vi "VIH Utility - FILE - List Directory Advanced.vi"(4 "Exclude Dir patterns":string[](array[string]), 6 "Exclude File patterns":string[](array[string]), 7 "List recursively (F)":bool, 8 "error in":errorcluster, 9 "Directory patterns":string[](array[string]), 10 "File patterns":string[](array[string]), 11 "directory path":path) -> (0 "error out":errorcluster, 1 "sub-directory paths":path[](array[path]), 2 "file paths":path[](array[path]), 3 "dup directory path":path)   [LabVIEW 2014]
doc: "::: VI Helpeks :::\nCopyright (c) 2000-2026 Konstantin Shifershteyn. All rights reserved."
panel:
  # "VI Helpeks\nCopyright (c) 2012-2026 Konstantin Shifershteyn"
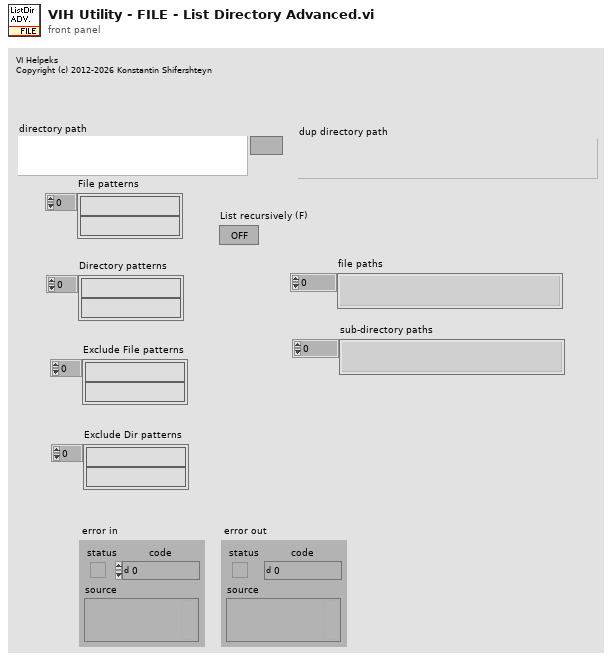
[diagram p1: front panel]
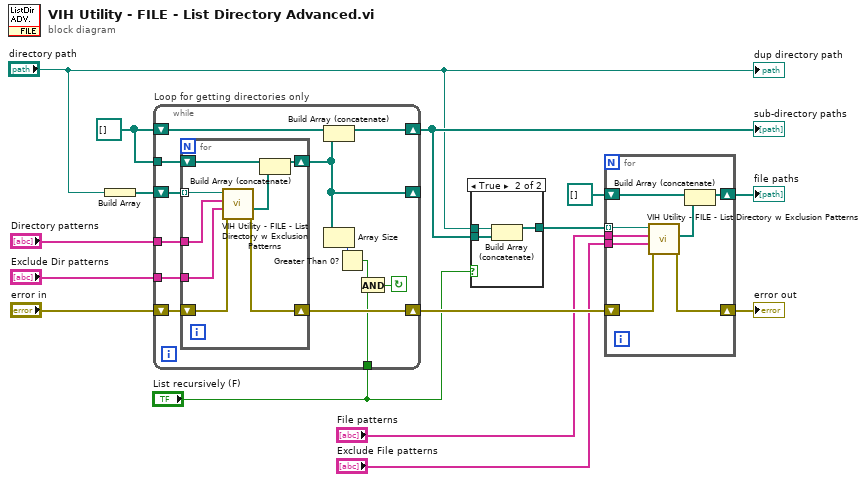
[diagram p0: block diagram]
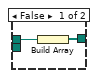
[diagram p2: hidden frame]
diagram:
  w15 = path[] []
  n1 = Build Array("directory path") -> (w14:path[])
  n2 = while "Loop for getting directories only" {
    tunnel: w15 -> [w24]
    shift-left: w15 -> [w28]
    shift-right: [w27] -> w10
    shift-left: "error in" -> [w22]
    shift-right: [w21] -> w8
    shift-left: w14 -> [w25]
    shift-right: [w23] -> _
    tunnel: "Directory patterns" -> [w20]
    tunnel: "Exclude Dir patterns" -> [w19]
    tunnel: "List recursively (F)" -> [w16]
    stop <- w18 continue-if-true
    n3 = for {
      tunnel: w25 -> [w36] mode=indexing
      shift-right: [w33] -> w23
      shift-left: w24 -> [w35]
      shift-right: [w31] -> w21
      shift-left: w22 -> [w32]
      tunnel: w20 -> [w30]
      tunnel: w19 -> [w29]
      n4 = call "VIH Utility - FILE - List Directory w Exclusion Patterns.vi"("error in"=w32, "Exclude patterns"=w29, "Include patterns"=w30, "directory path"=w36) -> ("error out"=w31:errorcluster, "directory paths"=w34:path[])  [unwired: 6 out]
      n5 = Build Array (concatenate)(w35, w34) -> (w33:path[])
    }
    n6 = Build Array (concatenate)(w28, w23) -> (w27:path[])
    n7 = Array Size(array=w23) -> (size(s)=w26:i32)
    n8 = Greater Than 0?(x=w26) -> (x > 0?=w17:bool)
    n9 = And(x=w17, y=w16) -> (x .and. y?=w18:bool)
  }
  "sub-directory paths" <- w10
  n10 = case shown="True" "List recursively (F)" {
    tunnel: w10 -> [_ w41]
    tunnel: [w38 w40] -> w3
    tunnel: "directory path" -> [w37 w39]
    frame False {
      n11 = Build Array(w37) -> (w38:path[])
    }
    frame True {
      n12 = Build Array (concatenate)(w39, w41) -> (w40:path[])
    }
  }
  n13 = for {
    tunnel: w3 -> [w49] mode=indexing
    shift-right: [w47] -> w6
    shift-left: path[] [] -> [w48]
    shift-right: [w44] -> w7
    shift-left: w8 -> [w45]
    tunnel: "File patterns" -> [w43]
    tunnel: "Exclude File patterns" -> [w42]
    n14 = call "VIH Utility - FILE - List Directory w Exclusion Patterns.vi"("error in"=w45, "Exclude patterns"=w42, "Include patterns"=w43, "directory path"=w49) -> ("error out"=w44:errorcluster, "file paths"=w46:path[])  [unwired: 6 out]
    n15 = Build Array (concatenate)(w48, w46) -> (w47:path[])
  }
  "error out" <- w7
  "file paths" <- w6
  "dup directory path" <- "directory path"
